vi "Flush Queue to File.vi"(8 "error in (no error)":errorcluster, 11 "Event Reporter Module in":refnum<class "Event Reporter Module.lvclass">) -> (0 "error out":errorcluster, 3 "Event Reporter Module out":refnum<class "Event Reporter Module.lvclass">)   [LabVIEW 2020, in "Volatus.lvlib" / "Event Reporter Module.lvclass"]
uses:
  Event Reporter Module.lvclass
  Event Reporter Module.lvclass/Event Reporter Module.ctl
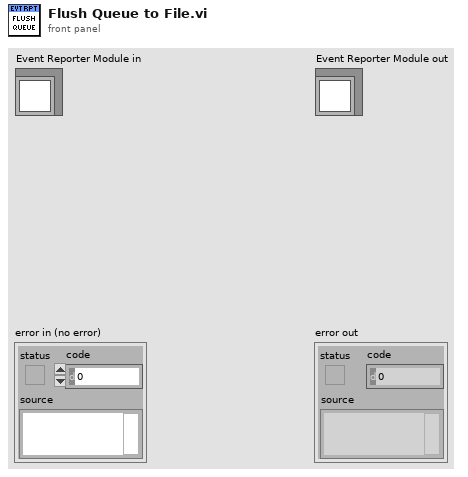
[diagram p1: front panel]
types:
  T1 = typedef "Volatus.lvlib/Event.ctl" = cluster{"Time Stamp":timestamp, "Event Level":T2, "Context":string, "Message":string, "Error":errorcluster, "Node":string}
  T2 = typedef "Volatus.lvlib/Event Level.ctl" = enum16{"Debug", "Info", "Warning", "Error"}
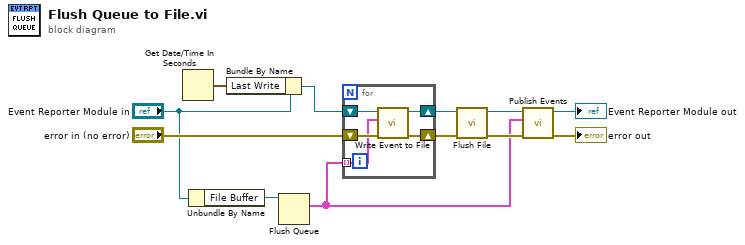
[diagram p0: block diagram]
diagram:
  n1 = Get Date/Time In Seconds() -> (seconds since 1Jan1904=w7:timestamp)
  n2 = Unbundle By Name("Event Reporter Module in") -> ("File Buffer"=w11:refnum<queue>)
  n3 = Bundle By Name(cluster="Event Reporter Module in", "Last Write"=w7) -> (w8:refnum<class "Event Reporter Module.lvclass">)
  n4 = Flush Queue(queue=w11) -> (remaining elements=w1:T1[])  [unwired: 1 in, 2 out]
  n5 = for {
    shift-right: [w14] -> w5
    shift-left: w8 -> [w17]
    shift-right: [w13] -> w9
    shift-left: "error in (no error)" -> [w16]
    tunnel: w1 -> [w15] mode=indexing
    n6 = call "Write Event to File.vi"("error in (no error)"=w16, "Event"=w15, "Event Reporter Module in"=w17) -> ("error out"=w13:errorcluster, "Event Reporter Module out"=w14:refnum<class "Event Reporter Module.lvclass">)  [unwired: 7 in]
  }
  n7 = call "Flush File.vi"("error in (no error)"=w9, "Event Reporter Module in"=w5) -> ("error out"=w6:errorcluster, "Event Reporter Module out"=w3:refnum<class "Event Reporter Module.lvclass">)  [unwired: 8 in]
  n8 = call "Publish Events.vi"("error in (no error)"=w6, "Events"=w1, "Event Reporter Module in"=w3) -> ("error out"=→"error out":errorcluster, "Event Reporter Module out"=→"Event Reporter Module out":refnum<class "Event Reporter Module.lvclass">)  [unwired: 7 in]
